vi "Send message to TCP Server.vi"(7 "LabVIEW Object":refnum<class>, 8 "error in (no error)":errorcluster, 10 "String":string, 11 "IP":string) -> (0 "error out":errorcluster)   [LabVIEW 2020, in "TALOS.lvlib"]
uses:
  TALOS.lvlib
  Ancestor/Ancestor/Ancestor.lvclass/Ancestor.ctl
  Generate Error.vi
  FGV/Error Memory/Get Error Description.vi
  Get PC name.vi
  Ancestor/Ancestor/Read ID.vi
  Get Class Name.vi
  <vilib>/Utility/error.llb/Clear Errors.vi
  FGV/Error Memory/Error Memory Core.vi
  <vilib>/AdvancedString/Delimited String to 1D String Array.vi
  Circus Root Path.vi
  FGV/Error Memory/Error Crt Lvl checker.vi
  FGV/Error Memory/Error Memory Core.vi/40c8088d-b597-4017-91af-faa98e00292e.vi
  FGV/Error Memory/Error Memory Core.vi/d4a3ab98-063c-4e44-b43d-fbdcfe6c2be2.vi
  Global Constants.vi
  Global Memory.vi
  <vilib>/Utility/LVClass/Get LV Class Name.vi
  Is in Packed Library.vi
  TALOS Root path.vi
  Read CSV worksheet.vi
  <vilib>/Utility/error.llb/General Error Handler.vi
  Error Log.vi
  Ancestor/Ancestor/Ancestor.lvclass
  <vilib>/Comparison/Equal/Equal Functor/Equal Functor.lvclass
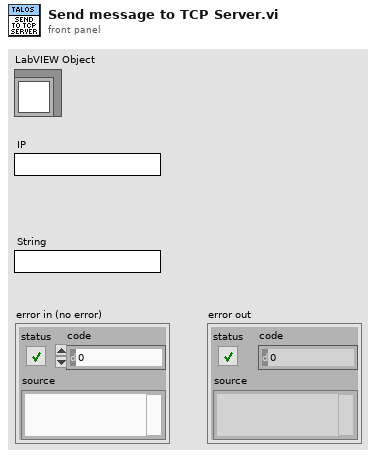
[diagram p1: front panel]
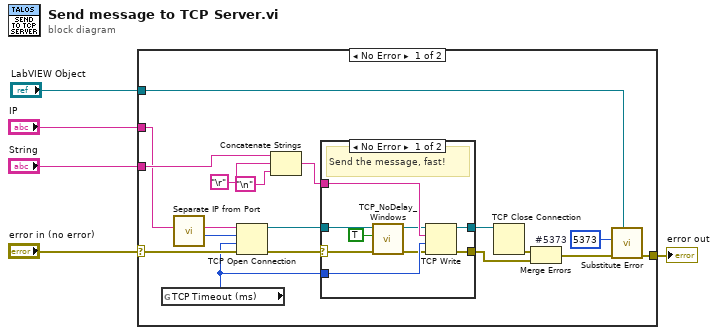
[diagram p0: block diagram]
diagram:
  n1 = case shown="No Error" "error in (no error)" {
    selector: "error in (no error)" -> [w14 w35]
    tunnel: "String" -> [w22 _]
    tunnel: "IP" -> [w8 _]
    tunnel: [w11 w35] -> w2
    tunnel: "LabVIEW Object" -> [w10 _]
    frame No Error {
      w13 = 5373  # #5373
      n2 = global read "Global Constants.vi" "TCP Timeout (ms)"() -> (w9:i32)
      n3 = call "Separate IP from Port.vi"("IP+Port"=w8) -> ("Port"=w6:u16, "IP"=w7:string)  [unwired: 9 in]
      n4 = TCP Open Connection(address=w7, remote port or service name=w6, timeout ms (60000)=w9, error in (no error)=w14) -> (connection ID=w18:refnum<k5>, error out=w17:errorcluster)  [unwired: 1 in]
      n5 = Concatenate Strings(w22, "\r", "\n") -> (w23:string)
      n6 = case shown="No Error" w17 {
        selector: w17 -> [w29 w33]
        tunnel: w9 -> [w32 _]
        tunnel: w23 -> [w31 _]
        tunnel: [w30 w34] -> w16
        tunnel: w18 -> [w26 w34]
        tunnel: [w24 w33] -> w19
        frame No Error {
          # "Send the message, fast!"
          n7 = call "TCP_NoDelay_Windows.vi"("error in (no error)"=w29, "TCP_NODELAY (true)"=TRUE, "connID"=w26) -> ("error out"=w28:errorcluster, "connID 2"=w27:refnum<k5>)  [unwired: 3 in]
          n8 = TCP Write(connection ID=w27, data in=w31, error in (no error)=w28, 9:w32) -> (connection ID out=w30:refnum<k5>, error out=w24:errorcluster)  [unwired: 1 out]
        }
        frame Error {
          # "Go straight to Close"
        }
      }
      n9 = TCP Close Connection(connection ID=w16) -> (error out=w15:errorcluster)  [unwired: 2 in, 1 out]
      n10 = Merge Errors(w15, w19) -> (w12:errorcluster)
      n11 = call "Substitute Error.vi"("LabVIEW Object"=w10, "error in (no error)"=w12, "Error Code"=w13) -> ("error out"=w11:errorcluster)  [unwired: 8 in]
    }
    frame Error {
    }
  }
  "error out" <- w2
